vi "Read CIF Publisher Info.vi"(8 "error in (no error)":errorcluster, 10 "CIF Subscriber Refnum":T2 {"refnum" format="%.0x"}, 11 "CIF Publisher Refnum":T1 {"refnum" format="%.0x"}) -> (0 "error out":errorcluster, 3 "CIF Publisher Info":T3)   [LabVIEW 2021, in "Iceoryx.lvlib"]
uses:
  Iceoryx.lvlib
  typedef/CIF Pcap Publisher Info.ctl
  SubVIs/Convert Error Core.vi
  Refnum/Typedef/CIF Subscriber Refnum.ctl
  Refnum/Typedef/CIF Publisher Refnum.ctl
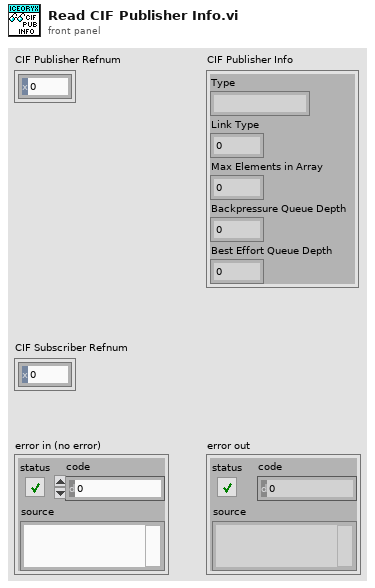
[diagram p1: front panel]
types:
  T1 = typedef "Iceoryx.lvlib/CIF Publisher Refnum.ctl" = cluster{"refnum":u64, "CIF Pub":enum8{"cifpub"}}
  T2 = typedef "Iceoryx.lvlib/CIF Subscriber Refnum.ctl" = cluster{"refnum":u64, "CIF Sub":enum8{"cifsub"}}
  T3 = typedef "Iceoryx.lvlib/CIF Pcap Publisher Info.ctl" = cluster{"Type":string, "Link Type":u32, "Max Elements in Array":u32, "Backpressure Queue Depth":u32, "Best Effort Queue Depth":u32}
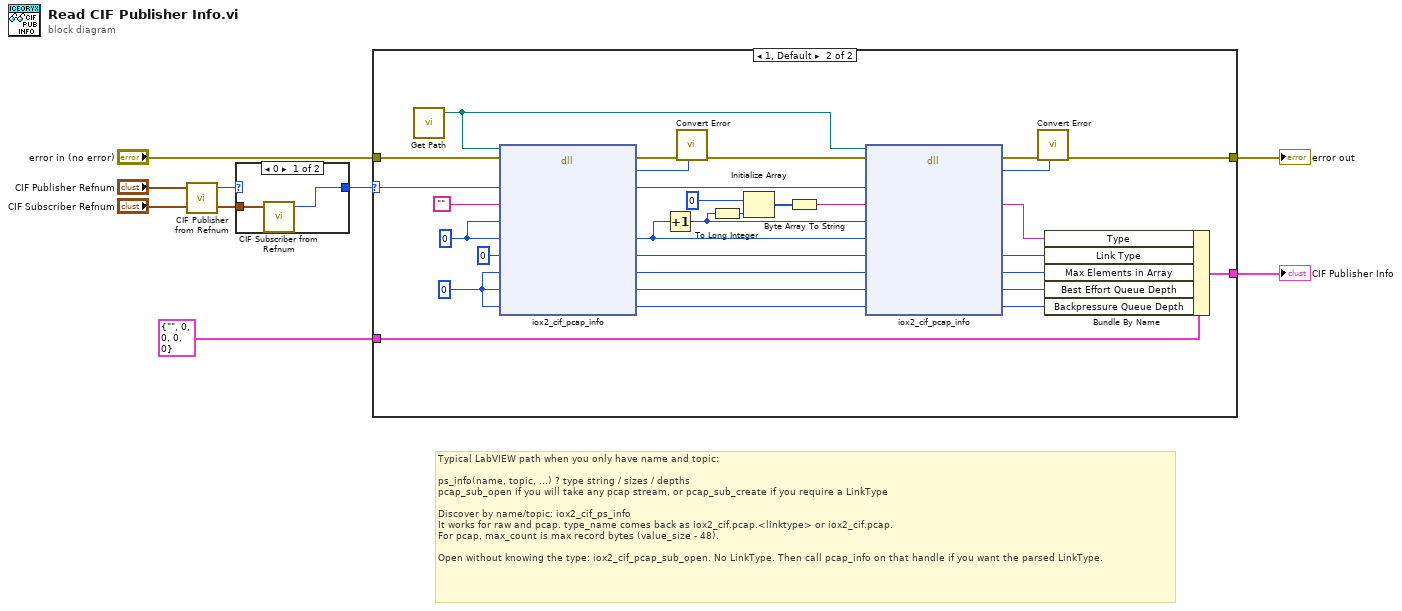
[diagram p0: block diagram]
diagram:
  # "Typical LabVIEW path when you only have name and topic:\n\nps_info(name, topic, …) ? type string / sizes / depths\npcap_sub_open if you will take any pcap stream, or pcap_sub_create if you require a LinkType\n\nDiscover by name/topic: iox2_cif_ps_info\nIt works for raw and pcap. type_name comes back as iox2_cif.pcap.<linktype> or iox2_cif.pcap. \nFor pcap, max_count is max record bytes (value_size - 48).\n\nOpen without knowing the type: iox2_cif_pcap_sub_open. No LinkType. Then call pcap_info on that handle if you want the parsed LinkType."
  n1 = call "CIF Publisher from Refnum.vi"("CIF Publisher Refnum"="CIF Publisher Refnum") -> ("CIF Publisher U64"=w2:u64)  [unwired: 4 in]
  n2 = case shown="0" w2 {
    selector: w2 -> [_ w11]
    tunnel: "CIF Subscriber Refnum" -> [w10 _]
    tunnel: [w9 w11] -> w1
    frame 0 {
      n3 = call "CIF Subscriber from Refnum.vi"("CIF Subscriber Refnum"=w10) -> ("CIF Subscriber U64"=w9:u64)  [unwired: 4 in]
    }
    frame 1, Default {
    }
  }
  n4 = case shown="1, Default" w1 {
    selector: w1 -> [_ w15]
    tunnel: "error in (no error)" -> [w12 w44]
    tunnel: [w12 w39] -> w7
    tunnel: [w13 w16] -> w6
    tunnel: T3 {"Type"="", "Link Type"=0, "Max Elements in Array"=0, "Backpressure Queue Depth"=0, "Best Effort Queue Depth"=0} ("CIF Publisher Info") -> [w13 w14]
    frame 0 {
    }
    frame 1, Default {
      w35 = u32 0 ("max_count")
      w41 = u32 0 ("actual")
      n5 = call "Get Path.vi"() -> ("libiox2_cif path"=w33:path)  [unwired: 4 in]
      n6 = dll-call lib="D:/dev/iceoryx2_lvwrapper/dist/iox2_cif.dll" fn="iox2_cif_pcap_info"(path in=w33, error in=w44, "port"=w15, "type_name"="", "type_cap"=w41, "type_len"=w41, "linktype"=u32 0, "max_cap_bytes"=w35, "be_subscriber_buffer"=w35, "bp_subscriber_buffer"=w35) -> (error out=w43:errorcluster, "return type"=w42:i32, "port"=w23:u64, "type_len"=w17:u32, "linktype"=w25:u32, "max_cap_bytes"=w28:u32, "be_subscriber_buffer"=w27:u32, "bp_subscriber_buffer"=w26:u32)  [unwired: 3 in, 1 out]
      n7 = Increment(x=w17) -> (x+1=w29:u32)
      n8 = call "Convert Error.vi"("return type"=w42, "error in (no error)"=w43) -> ("error out"=w34:errorcluster)  [unwired: 9 in]
      n9 = To Long Integer(number=w29) -> (32bit integer=w37:i32)
      n10 = Initialize Array(u8 0 ("actual"), w37) -> (w36:u8[])
      n11 = Byte Array To String(unsigned byte array=w36) -> (string=w30:string)
      n12 = dll-call lib="D:/dev/iceoryx2_lvwrapper/dist/iox2_cif.dll" fn="iox2_cif_pcap_info"(path in=w33, error in=w34, "port"=w23, "type_name"=w30, "type_cap"=w29, "type_len"=w17, "linktype"=w25, "max_cap_bytes"=w28, "be_subscriber_buffer"=w27, "bp_subscriber_buffer"=w26) -> (error out=w32:errorcluster, "return type"=w31:i32, "type_name"=w22:string, "linktype"=w18:u32, "max_cap_bytes"=w21:u32, "be_subscriber_buffer"=w19:u32, "bp_subscriber_buffer"=w20:u32)  [unwired: 4 in, 1 out]
      n13 = call "Convert Error.vi"("return type"=w31, "error in (no error)"=w32) -> ("error out"=w39:errorcluster)  [unwired: 9 in]
      n14 = Bundle By Name(cluster=w14, "Type"=w22, "Link Type"=w18, "Max Elements in Array"=w21, "Best Effort Queue Depth"=w19, "Backpressure Queue Depth"=w20) -> (w16:T3)
    }
  }
  "error out" <- w7
  "CIF Publisher Info" <- w6
